vi "VIH HelpGen - Create Wrapper VI - Code & ConPane.vi"(8 "error in":errorcluster, 9 "Terminal Wiring Rules":u16[](array[numeric]), 10 "Target VI Refnum":refnum<vi>, 11 "Source VI Refnum":refnum<vi>) -> (0 "error out":errorcluster, 2 "dup Target VI Refnum":refnum<vi>, 3 "dup Source VI Refnum":refnum<vi>)   [LabVIEW 2014]
doc: "::: VI Helpeks :::\nCopyright (c) 2000-2026 Konstantin Shifershteyn. All rights reserved."
uses:
  <vilib>/Utility/miscctls.llb/LVPointTypeDef.ctl
panel:
  # "VI Helpeks\nCopyright (c) 2012-2026 Konstantin Shifershteyn"
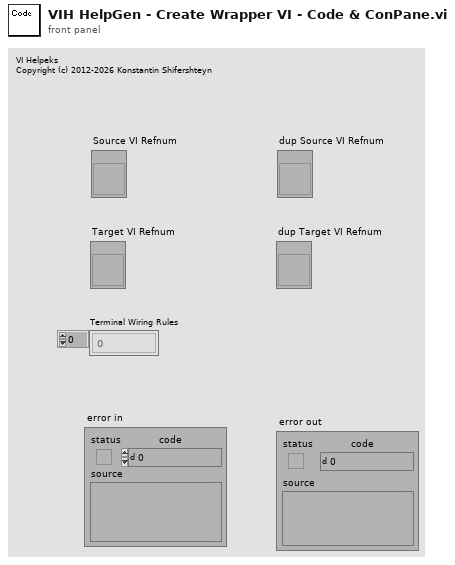
[diagram p1: front panel]
types:
  T1 = typedef "LVPointTypeDef.ctl" = cluster{"Horizontal":i16, "Vertical":i16}
  T2 = cluster{"IsSource":bool, i32, refnum<vi>, "Name":string}
  T3 = cluster{"IsSource":bool, i32, refnum<vi>, "Name":string}[]
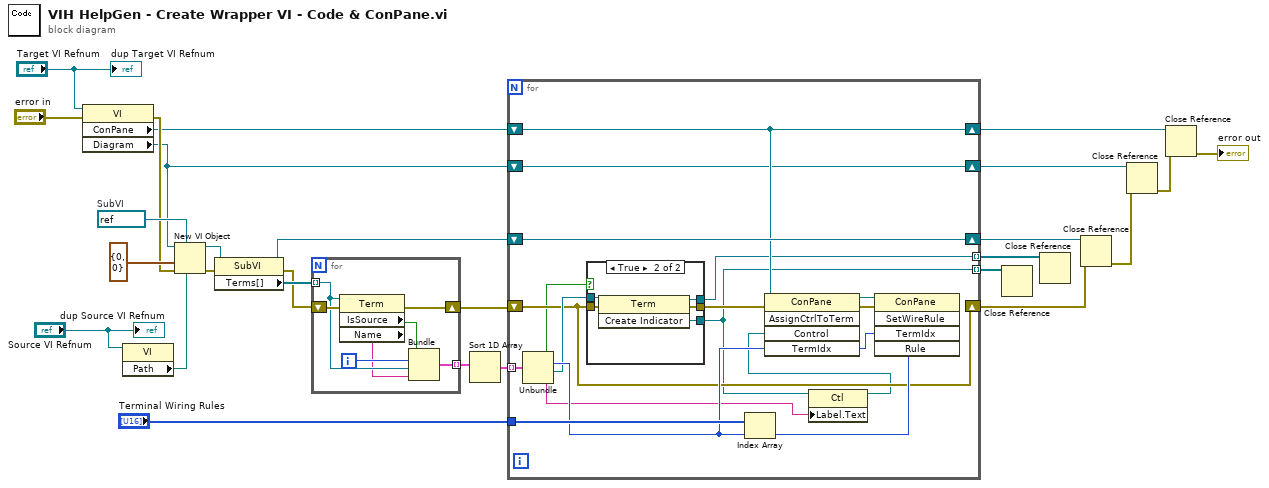
[diagram p0: block diagram]
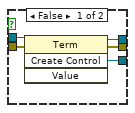
[diagram p2: hidden frame]
diagram:
  w27 = refnum<vi> refnum  # SubVI
  n1 = property class="VI"(reference="Target VI Refnum", error in="error in") -> (error out=w22:errorcluster, "ConPane"=w15:refnum<vi>, "Diagram"=w13:refnum<vi>)  [unwired: 1 out]
  n2 = property class="VI"(reference="Source VI Refnum") -> ("Path"=w20:path)  [unwired: 1 in, 2 out]
  n3 = New VI Object(vi object class=w27, owner refnum=w13, position/next to=T1 {"Horizontal"=0, "Vertical"=0} ("location"), 6:w20, 8:w22) -> (object refnum=w25:refnum<vi>, 0:w17:errorcluster)  [unwired: 3 in]
  n4 = property class="SubVI"(reference=w25, error in=w17) -> (reference out=w16:refnum<vi>, error out=w23:errorcluster, "Terms[]"=w24:refnum<vi>[])
  n5 = for {
    tunnel: w24 -> [w29] mode=indexing
    shift-right: [w31] -> w9
    shift-left: w23 -> [w32]
    tunnel: [w30] -> w10 mode=indexing
    i -> [w33]
    n6 = property class="Term"(reference=w29, error in=w32) -> (error out=w31:errorcluster, "IsSource"=w34:bool, "Name"=w28:string)  [unwired: 1 out]
    n7 = Bundle("IsSource"=w34, w33, w29, "Name"=w28) -> (w30:T2)  [unwired: 1 in]
  }
  n8 = Sort 1D Array(array=w10) -> (sorted array=w11:T3)
  n9 = for {
    shift-right: [w39] -> w6
    shift-left: w9 -> [w39]
    shift-right: [w50] -> w1
    shift-left: w16 -> [w50]
    shift-right: [w49] -> w2
    shift-left: w15 -> [w49]
    shift-right: [w48] -> w5
    shift-left: w13 -> [w48]
    tunnel: "Terminal Wiring Rules" -> [w45]
    tunnel: [w43] -> w7 mode=indexing
    tunnel: [w37] -> w8 mode=indexing
    tunnel: w11 -> [w42] mode=indexing
    n10 = Unbundle(w42) -> ("IsSource"=w38:bool, w41:i32, w40:refnum<vi>, "Name"=w36:string)
    n11 = case shown="True" w38 {
      tunnel: [w56 w61] -> w51
      tunnel: w40 -> [w55 w60]
      tunnel: w39 -> [w54 w59]
      tunnel: [w53 w58] -> w37
      tunnel: [w52 w57] -> w43
      frame False {
        n12 = invoke class="Term" method="Create Control"(reference=w55, error in=w54) -> (reference out=w52:refnum<vi>, error out=w56:errorcluster, "Create Control"=w53:refnum<vi>)  [unwired: 2 in, 1 out]
      }
      frame True {
        n13 = invoke class="Term" method="Create Indicator"(reference=w60, error in=w59) -> (reference out=w57:refnum<vi>, error out=w61:errorcluster, "Create Indicator"=w58:refnum<vi>)  [unwired: 1 in]
      }
    }
    n14 = Index Array(array=w45, index=w41) -> (element=w44:u16)
    n15 = property class="Ctl"(reference=w37, "Label.Text"=w36) -> (reference out=w35:refnum<vi>)  [unwired: 1 in, 1 out]
    n16 = invoke class="ConPane" method="AssignCtrlToTerm"(reference=w49, error in=w51, "Control"=w35, "TermIdx"=w41) -> (reference out=w47:refnum<vi>, error out=w46:errorcluster)  [unwired: 1 in, 3 out]
    n17 = invoke class="ConPane" method="SetWireRule"(reference=w47, error in=w46, "TermIdx"=w41, "Rule"=w44) -> ()  [unwired: 1 in, 5 out]
  }
  n18 = Close Reference(reference=w8) -> ()  [unwired: 1 in, 1 out]
  n19 = Close Reference(reference=w7) -> ()  [unwired: 1 in, 1 out]
  n20 = Close Reference(reference=w1, error in (no error)=w6) -> (error out=w3:errorcluster)
  n21 = Close Reference(reference=w5, error in (no error)=w3) -> (error out=w4:errorcluster)
  n22 = Close Reference(reference=w2, error in (no error)=w4) -> (error out=→"error out":errorcluster)
  "dup Source VI Refnum" <- "Source VI Refnum"
  "dup Target VI Refnum" <- "Target VI Refnum"
